vi "TDMS_Write_Log.vi"(0 "File Path":path, 5 "Scaled Data":dbl[][](array[numeric]), 7 "Channels":T1(array[cluster]), 11 "error in":errorcluster) -> (15 "error out":errorcluster)   [LabVIEW 2026]
doc: "Channels[i].Save = True 인 채널만 TDMS 'AI Data' 그룹에 채널 이름(Name)으로 추가 기록(열기-쓰기-닫기)."
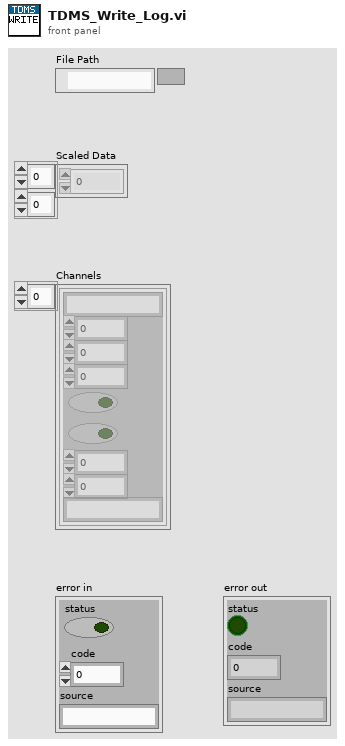
[diagram p1: front panel]
types:
  T1 = cluster{"Name":string, "Value":dbl, "High Limit":dbl, "Low Limit":dbl, "Save":bool, "Graph":bool, "Scale Min":dbl, "Scale Max":dbl, "Unit":string}[]
  T2 = enum16{"open", "open or create", "create or replace", "create", "open (read-only)"}
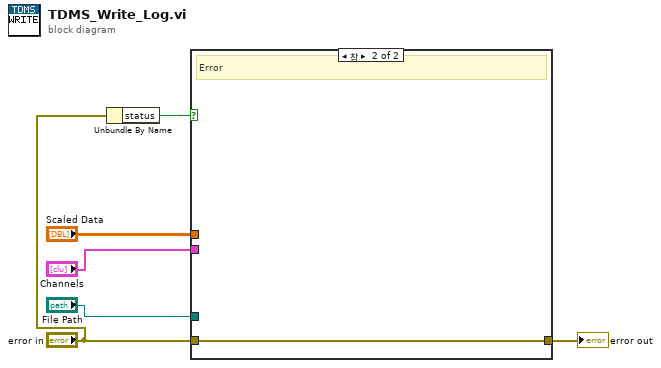
[diagram p0: block diagram]
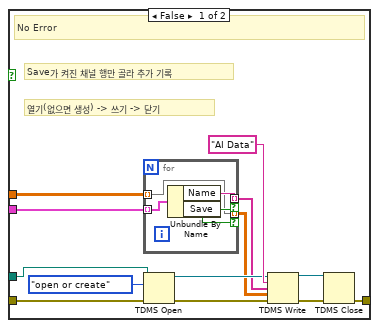
[diagram p2: hidden frame]
diagram:
  n1 = Unbundle By Name("error in") -> ("status"=w5:bool)
  n2 = case shown="참" w5 {
    tunnel: "File Path" -> [w7 _]
    tunnel: "Scaled Data" -> [w8 _]
    tunnel: "Channels" -> [w9 _]
    tunnel: "error in" -> [w10 w24]
    tunnel: [w19 w24] -> w6
    frame False {
      # "열기(없으면 생성) -> 쓰기 -> 닫기"
      # "Save가 켜진 채널 행만 골라 추가 기록"
      # "No Error"
      n3 = for {
        tunnel: w8 -> [w20] mode=indexing
        tunnel: w9 -> [w21] mode=indexing
        tunnel: [w20] -> w11 mode=indexing if=w23
        tunnel: [w22] -> w12 mode=indexing if=w23
        n4 = Unbundle By Name(w21) -> ("Name"=w22:string, "Save"=w23:bool)
      }
      n5 = TDMS Open(8:w10, 10:T2."open or create", 11:w7) -> (0:w15:errorcluster, 3:w14:refnum<k34>)  [unwired: 4 in]
      n6 = TDMS Write(0:w14, 5:"AI Data", 7:w12, 9:w11, 11:w15) -> (4:w17:refnum<k34>, 15:w18:errorcluster)  [unwired: 1 in, 2 out]
      n7 = TDMS Close(8:w18, 11:w17) -> (0:w19:errorcluster)  [unwired: 1 out]
    }
    frame True {
      # "Error"
    }
  }
  "error out" <- w6
